vi "Test Reverse String.vi"(8 "error in (no error)":errorcluster) -> (0 "error out":errorcluster, 3 "Pass?":bool)   [LabVIEW 2020]
uses:
  G-Unicode/Unicode/Controls/String Encoding.ctl
  G-Unicode/Types/UTF-8 String/UTF-8 String.lvclass/UTF-8 String.ctl
  95d7db13-e1eb-4656-9a00-7ce04d3ddba8.vi
  8690b08d-f36c-4ee5-acde-790fa2950b16.vi
  ba5b6683-6b7f-4241-8972-fb5dd34213e6.vi
  504d7c14-23e1-4c14-92bf-7573e680de72.vi
  422f9b4b-c10b-46b7-b73f-1268a1c43e11.vi
  239b2762-dc91-42b6-b8b8-d649fddcbd19.vi
  G-Unicode/Unicode/Encode String.vi
  95d7db13-e1eb-4656-9a00-7ce04d3ddba8.vi/46bf550a-28c6-4dfd-813a-9b0ad34779ef.vi
  G-Unicode/Private/Conversion/String as Encoded String.vi
  G-Unicode/Private/Conversion/Polymorphic VIs/String as Encoded String (UTF-8 String).vi
  G-Unicode/Types/UTF-8 String/Write Encoded UTF-8 String.vi
  G-Unicode/Private/Conversion/Polymorphic VIs/String as Encoded String (LabVIEW String).vi
  G-Unicode/Private/Library/gu_reverse_string.vi
  ba5b6683-6b7f-4241-8972-fb5dd34213e6.vi/3a31b270-3bb6-4c58-a256-c5fcc2c98f09.vi
  ba5b6683-6b7f-4241-8972-fb5dd34213e6.vi/0ec5df2d-ef9b-4f84-a6a8-ffcedd45c4dc.vi
  239b2762-dc91-42b6-b8b8-d649fddcbd19.vi/3a31b270-3bb6-4c58-a256-c5fcc2c98f09.vi
  239b2762-dc91-42b6-b8b8-d649fddcbd19.vi/0ec5df2d-ef9b-4f84-a6a8-ffcedd45c4dc.vi
  G-Unicode/Private/Conversion/Text to UTF-8.vi
  G-Unicode/Private/Conversion/Polymorphic VIs/Text to UTF-8 (LabVIEW String).vi
  G-Unicode/Private/Conversion/Encoded UTF-8 String to Encoded UTF-16LE String.vi
  G-Unicode/Unicode/SubVIs/UTF-16 Byte Swap.vi
  G-Unicode/Private/Conversion/UTF-8 to Text.vi
  G-Unicode/Private/Conversion/Polymorphic VIs/UTF-8 to Text (LabVIEW String).vi
  G-Unicode/Private/Conversion/Encoded UTF-16LE String to Encoded UTF-8 String.vi
  G-Unicode/Unicode/Prepend BOM.vi
  G-Unicode/Types/UTF-8 String/Read Encoded UTF-8 String.vi
  G-Unicode/Private/Library/Result To Error.vi
  G-Unicode/Private/Conversion/Text as Encoded String.vi
  G-Unicode/Private/Conversion/Polymorphic VIs/Text as Encoded String (LabVIEW String).vi
  G-Unicode/Private/Conversion/Polymorphic VIs/Text as Encoded String (UTF-8 String).vi
  G-Unicode/Unicode/SubVIs/Byte Order Marks.vi
  G-Unicode/Unicode/Detect BOM.vi
  <vilib>/Utility/error.llb/Error Cluster From Error Code.vi
  G-Unicode/Unicode/Detect String Encoding.vi
  G-Unicode/Types/UTF-8 String/UTF-8 String.lvclass
  G-Unicode/G-Unicode.lvlib
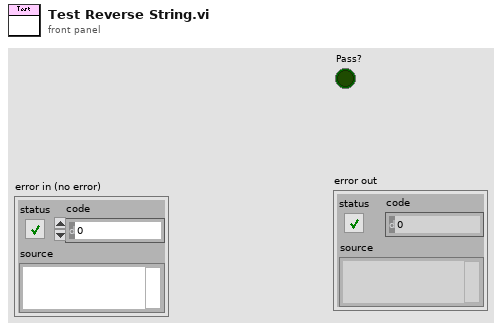
[diagram p1: front panel]
types:
  T1 = typedef "G-Unicode.lvlib/String Encoding.ctl" = enum16{"ANSI", "UTF-8", "UTF-16LE", "UTF-16BE", "Unknown"}
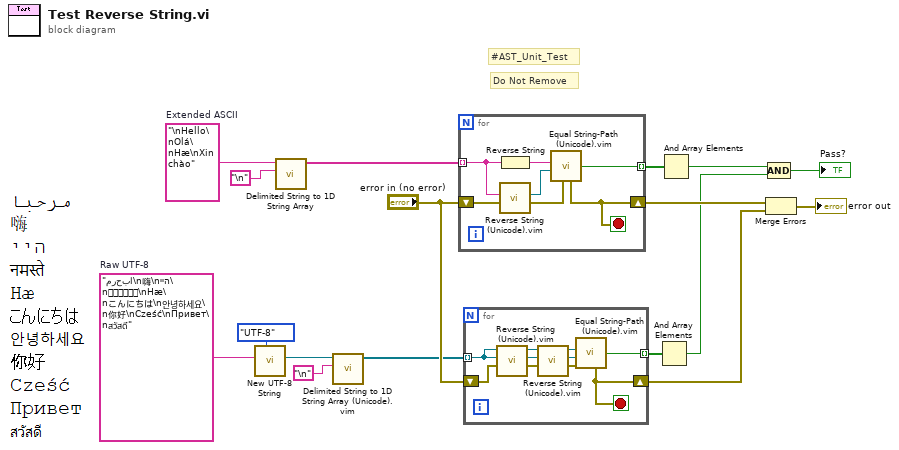
[diagram p0: block diagram]
diagram:
  w7 = "\nHello\nOlá\nHæ\nXin chào"  # Extended ASCII
  w3 = "مرحبا\n嗨\nהיי\nनमस्ते\nHæ\nこんにちは\n안녕하세요\n你好\nCześć\nПривет\nสวัสดี"  # Raw UTF-8
  # "Do Not Remove"
  # "#AST_Unit_Test"
  n1 = call "New UTF-8 String.vi"("Input Encoding (ANSI)"=String_Encoding."UTF-8", "String"=w3) -> ("UTF-8 String"=w2:refnum<class "UTF-8 String.lvclass">)  [unwired: 8 in, 1 out]
  n2 = call <vilib>:"Delimited String to 1D String Array.vi"("delimiter"="\n", "delimited string"=w7) -> ("string array"=w6:string[])  [unwired: 9 in]
  n3 = call "Delimited String to 1D String Array (Unicode).vim"("Delimiter (tab)"="\n", "Delimited String"=w2) -> ("String Array"=w4:refnum<class "UTF-8 String.lvclass">[])  [unwired: 8 in, 1 out]
  n4 = for {
    tunnel: [w24] -> w14 mode=indexing
    shift-right: [w18] -> w17
    shift-left: "error in (no error)" -> [w21]
    tunnel: w6 -> [w22] mode=indexing
    stop <- w18 stop-if-true
    n5 = Reverse String(1:w22) -> (0:w23:string)
    n6 = call "Reverse String (Unicode).vim"("error in"=w21, "String"=w22) -> ("error out"=w19:errorcluster, "Reversed"=w20:refnum<class "UTF-8 String.lvclass">)  [unwired: 8 in]
    n7 = call "Equal String-Path (Unicode).vim"("error in"=w19, "y"=w20, "x"=w23) -> ("error out"=w18:errorcluster, "Equal?"=w24:bool)  [unwired: 6 in]
  }
  n8 = for {
    tunnel: w4 -> [w29] mode=indexing
    tunnel: [w32] -> w12 mode=indexing
    shift-right: [w25] -> w10
    shift-left: "error in (no error)" -> [w28]
    stop <- w25 stop-if-true
    n9 = call "Reverse String (Unicode).vim"("error in"=w28, "String"=w29) -> ("error out"=w27:errorcluster, "Reversed"=w31:refnum<class "UTF-8 String.lvclass">)  [unwired: 8 in]
    n10 = call "Reverse String (Unicode).vim"("error in"=w27, "String"=w31) -> ("error out"=w26:errorcluster, "Reversed"=w30:refnum<class "UTF-8 String.lvclass">)  [unwired: 8 in]
    n11 = call "Equal String-Path (Unicode).vim"("error in"=w26, "y"=w30, "x"=w29) -> ("error out"=w25:errorcluster, "Equal?"=w32:bool)  [unwired: 6 in]
  }
  n12 = And Array Elements(Boolean array=w12) -> (logical AND=w11:bool)
  n13 = And Array Elements(Boolean array=w14) -> (logical AND=w13:bool)
  n14 = Merge Errors(w17, w10) -> (→"error out":errorcluster)
  n15 = Compound Arithmetic op=AND(w13, w11) -> (→"Pass?":bool)
